vi "Audio_Block.vi"(0 "Channels":T2, 1 "Sound":bool=TRUE, 5 "Bank":cluster{"Y":dbl[]}[](array[cluster]), 7 "Task ID":u32, 9 "Mixer":T1={"Current"=[], "Position"=0, "Priority"=99, "Music"=FALSE, "MusicPos"=0}, 11 "error in":errorcluster) -> (4 "Mixer out":T1={"Current"=[], "Position"=0, "Priority"=99, "Music"=FALSE, "MusicPos"=0}, 6 "Stop":bool, 15 "error out":errorcluster)   [LabVIEW 2020, in "GH_App.lvlib"]
doc: "One audio block: collects all sound bits from the sound queue, mixes 512 samples with Sound_Mix and writes them to the sound channel. Writing waits for room in the buffer - this paces the audio loop. Stop on an error (queue released = end of the game)."
uses:
  GH_App.lvlib
  Audio/GH_Audio.lvlib
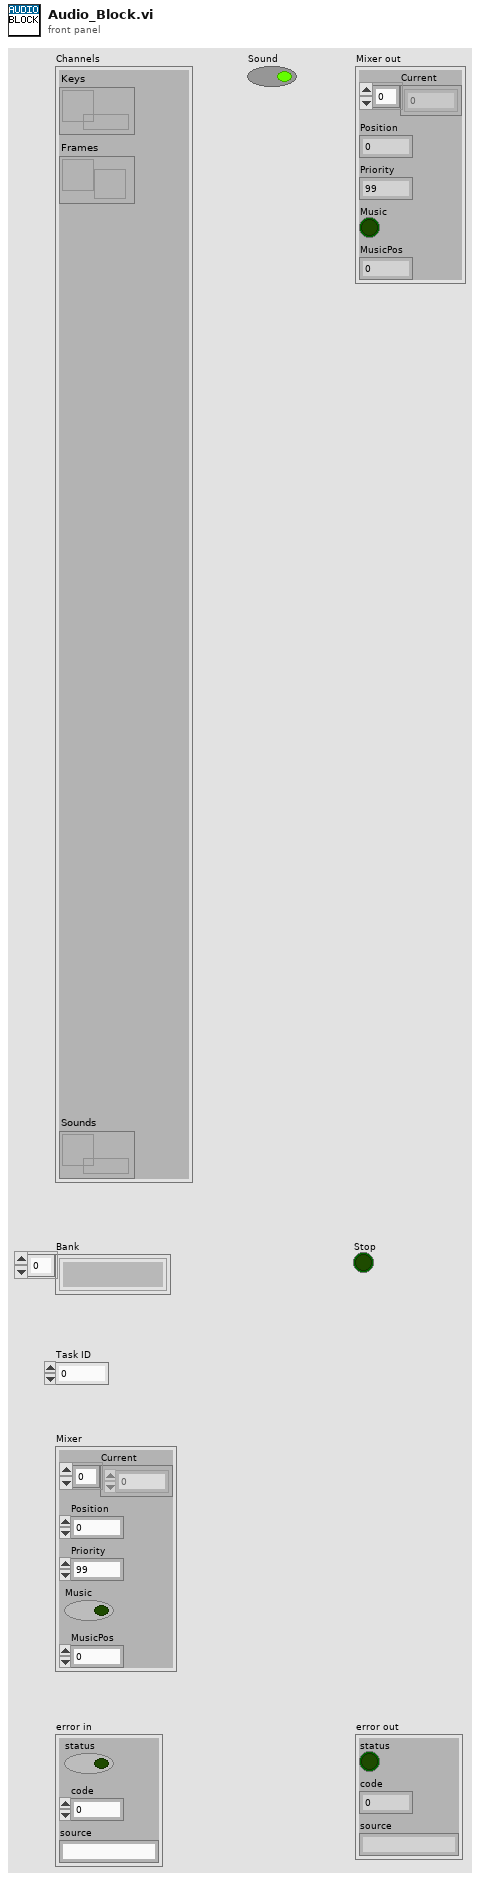
[diagram p1: front panel]
types:
  T1 = cluster{"Current":dbl[], "Position":i32, "Priority":i32, "Music":bool, "MusicPos":i32}
  T2 = cluster{"Keys":refnum<queue>, "Frames":refnum<notifier>, "Sounds":refnum<queue>}
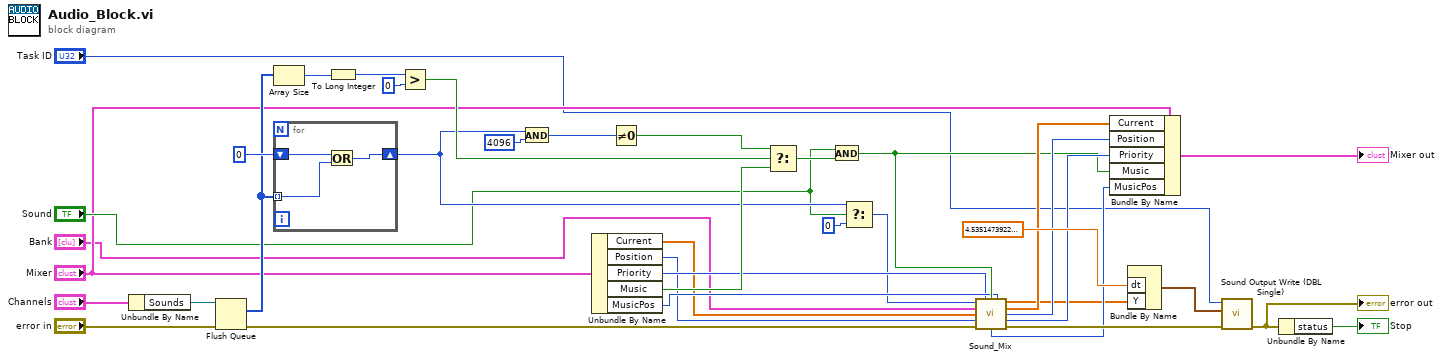
[diagram p0: block diagram]
diagram:
  n1 = Unbundle By Name("Channels") -> ("Sounds"=w7:refnum<queue>)
  n2 = Flush Queue(queue=w7, error in (no error)="error in") -> (remaining elements=w8:i32[], error out=w9:errorcluster)  [unwired: 1 out]
  n3 = Array Size(array=w8) -> (size(s)=w19:i32)
  n4 = for {
    shift-right: [w41] -> w11
    shift-left: 0 -> [w40]
    tunnel: w8 -> [w39] mode=indexing
    n5 = Or(x=w40, y=w39) -> (x .or. y?=w41:i32)
  }
  n6 = To Long Integer(number=w19) -> (32bit integer=w20:i32)
  n7 = Greater?(x=w20, y=0) -> (0:w22:bool)
  n8 = And(x=w11, y=4096) -> (x .and. y?=w24:i32)
  n9 = Unbundle By Name("Mixer") -> ("Current"=w14:dbl[], "Position"=w15:i32, "Priority"=w16:i32, "Music"=w17:bool, "MusicPos"=w18:i32)
  n10 = Not Equal To 0?(x=w24) -> (x != 0?=w25:bool)
  n11 = Select(t=w25, s=w22, f=w17) -> (s? t:f=w26:bool)
  n12 = And(x="Sound", y=w26) -> (x .and. y?=w27:bool)
  n13 = Select(t=w11, s="Sound", f=0) -> (s? t:f=w13:i32)
  n14 = call "Sound_Mix.vi"("Sounds"=w13, "Priority"=w16, "Music on"=w27, "Music Position"=w18, "Bank"="Bank", "Current"=w14, "Position"=w15, "error in"=w9) -> ("Block"=w28:dbl[], "Current out"=w29:dbl[], "Position out"=w30:i32, "Priority out"=w31:i32, "Music Position out"=w32:i32, "error out"=w33:errorcluster)  [unwired: 2 in]
  n15 = Bundle By Name(cluster="Mixer", "Current"=w29, "Position"=w30, "Priority"=w31, "Music"=w27, "MusicPos"=w32) -> (→"Mixer out":T1)
  n16 = Bundle By Name("dt"=4.5351473922902495e-05, "Y"=w28) -> (w35:waveform(dbl))  [unwired: 1 in]
  n17 = call <vilib>:"Sound Output Write (DBL Single).vi"("error in (no error)"=w33, "data"=w35, "task ID"="Task ID") -> ("error out"=w36:errorcluster)  [unwired: 7 in, 1 out]
  "error out" <- w36
  n18 = Unbundle By Name(w36) -> ("status"=→"Stop":bool)
